vi "Configure Resistor Band Visibility.vi"(8 "error in (no error)":errorcluster, 10 "Number of Bands in":T2=4 min=3 max=6 step=1, 11 "Color Refn":T1) -> (0 "error out":errorcluster, 2 "Number of Bands out":T2=4 min=3 max=6 step=1)   [LabVIEW 2018, in "Front Panel Interface.lvlib"]
doc: "Configures the visibility of the resistor band ColorBox controls on the Front Panel according to the selected number of bands.\n\nThe VI receives the <b>Number of Bands</b> and a cluster of <b>Color Refn</b>. It determines which resistor bands must be visible for 3-, 4-, 5-, and 6-band resistor configurations and updates the <b>Visible</b> property of each ColorBox control. <b>Number of Bands out</b> passes through the value of <b>Number of Bands in</b>.\n\nThe VI only configures Front Panel visibility. It does not modify the color or value of any resistor band."
uses:
  Front Panel Interface.lvlib
  Number of Bands--numeric.ctl
  Resistance Colors/Colors Refnums--cluster.ctl
  Resistance Colors/Resistance Colors.lvlib
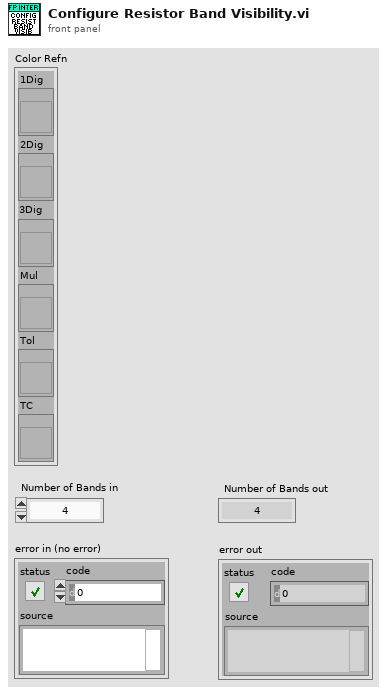
[diagram p1: front panel]
types:
  T1 = typedef "Resistance Colors.lvlib/Colors Refnums--cluster.ctl" = cluster{"1Dig":refnum<vi>, "2Dig":refnum<vi>, "3Dig":refnum<vi>, "Mul":refnum<vi>, "Tol":refnum<vi>, "TC":refnum<vi>}
  T2 = typedef "Number of Bands--numeric.ctl" = u8
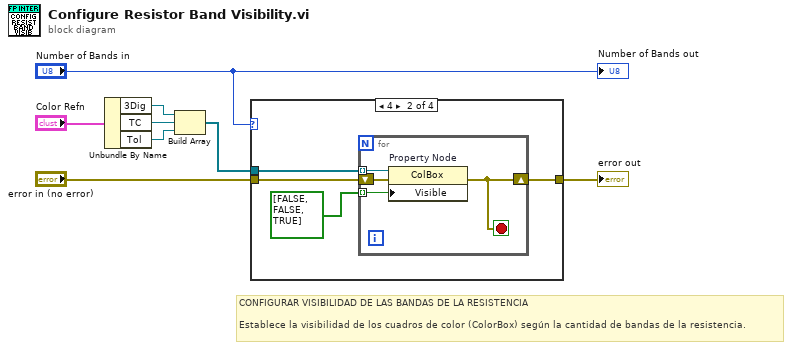
[diagram p0: block diagram]
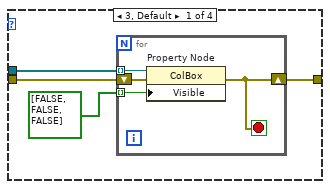
[diagram p2: hidden frame]
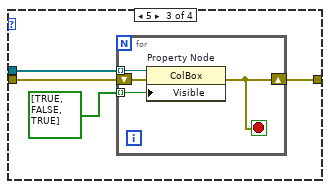
[diagram p3: hidden frame]
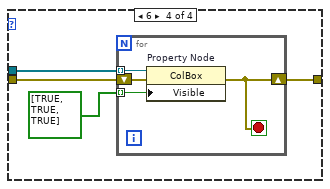
[diagram p4: hidden frame]
diagram:
  # "CONFIGURAR VISIBILIDAD DE LAS BANDAS DE LA RESISTENCIA\n\nEstablece la visibilidad de los cuadros de color (ColorBox) según la cantidad de bandas de la resistencia."
  n1 = Unbundle By Name("Color Refn") -> ("3Dig"=w3:refnum<vi>, "TC"=w4:refnum<vi>, "Tol"=w2:refnum<vi>)
  n2 = Build Array(w3, w4, w2) -> (w1:refnum<vi>[])
  n3 = case shown="4" "Number of Bands in" {
    tunnel: w1 -> [w12 w17 w28 w36]
    tunnel: [w10 w18 w25 w33] -> w8
    tunnel: "error in (no error)" -> [w9 w19 w26 w34]
    frame 3, Default {
      n4 = for {
        tunnel: w12 -> [w16] mode=indexing
        tunnel: bool[] [FALSE, FALSE, FALSE] -> [w15] mode=indexing
        shift-right: [w13] -> w10
        shift-left: w9 -> [w14]
        stop <- w13 stop-if-true
        n5 = property on="Property Node" class="ColBox"(reference=w16, error in=w14, "Visible"=w15) -> (error out=w13:errorcluster)  [unwired: 1 out]
      }
    }
    frame 4 {
      n6 = for {
        tunnel: w17 -> [w24] mode=indexing
        tunnel: bool[] [FALSE, FALSE, TRUE] -> [w23] mode=indexing
        shift-right: [w21] -> w18
        shift-left: w19 -> [w22]
        stop <- w21 stop-if-true
        n7 = property on="Property Node" class="ColBox"(reference=w24, error in=w22, "Visible"=w23) -> (error out=w21:errorcluster)  [unwired: 1 out]
      }
    }
    frame 5 {
      n8 = for {
        tunnel: w28 -> [w32] mode=indexing
        tunnel: bool[] [TRUE, FALSE, TRUE] -> [w31] mode=indexing
        shift-right: [w29] -> w25
        shift-left: w26 -> [w30]
        stop <- w29 stop-if-true
        n9 = property on="Property Node" class="ColBox"(reference=w32, error in=w30, "Visible"=w31) -> (error out=w29:errorcluster)  [unwired: 1 out]
      }
    }
    frame 6 {
      n10 = for {
        tunnel: w36 -> [w40] mode=indexing
        tunnel: bool[] [TRUE, TRUE, TRUE] -> [w39] mode=indexing
        shift-right: [w37] -> w33
        shift-left: w34 -> [w38]
        stop <- w37 stop-if-true
        n11 = property on="Property Node" class="ColBox"(reference=w40, error in=w38, "Visible"=w39) -> (error out=w37:errorcluster)  [unwired: 1 out]
      }
    }
  }
  "error out" <- w8
  "Number of Bands out" <- "Number of Bands in"
